vi "Command.vi"(8 "error in (no error)":errorcluster, 9 "command data":u8[](array[numeric]), 10 "node address":u8, 11 "ProPar in":refnum<class "PL Bronkhorst ProPar.lvclass">) -> (0 "error out":errorcluster, 2 "response data":u8[](array[numeric]), 3 "ProPar out":refnum<class "PL Bronkhorst ProPar.lvclass">)   [LabVIEW 2015, in "PL Bronkhorst ProPar.lvclass"]
doc: "Sends specified <b>command data</b> to specified <b>node</b> and returns <b>response data</b>."
uses:
  PL Bronkhorst ProPar.lvclass
  PL Bronkhorst ProPar.lvclass/PL Bronkhorst ProPar.ctl
panel:
  out "response":u8[](array[numeric])
  out "header":u8[](array[numeric])
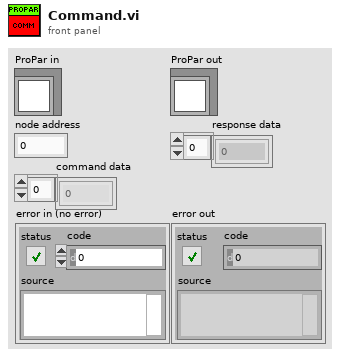
[diagram p1: front panel]
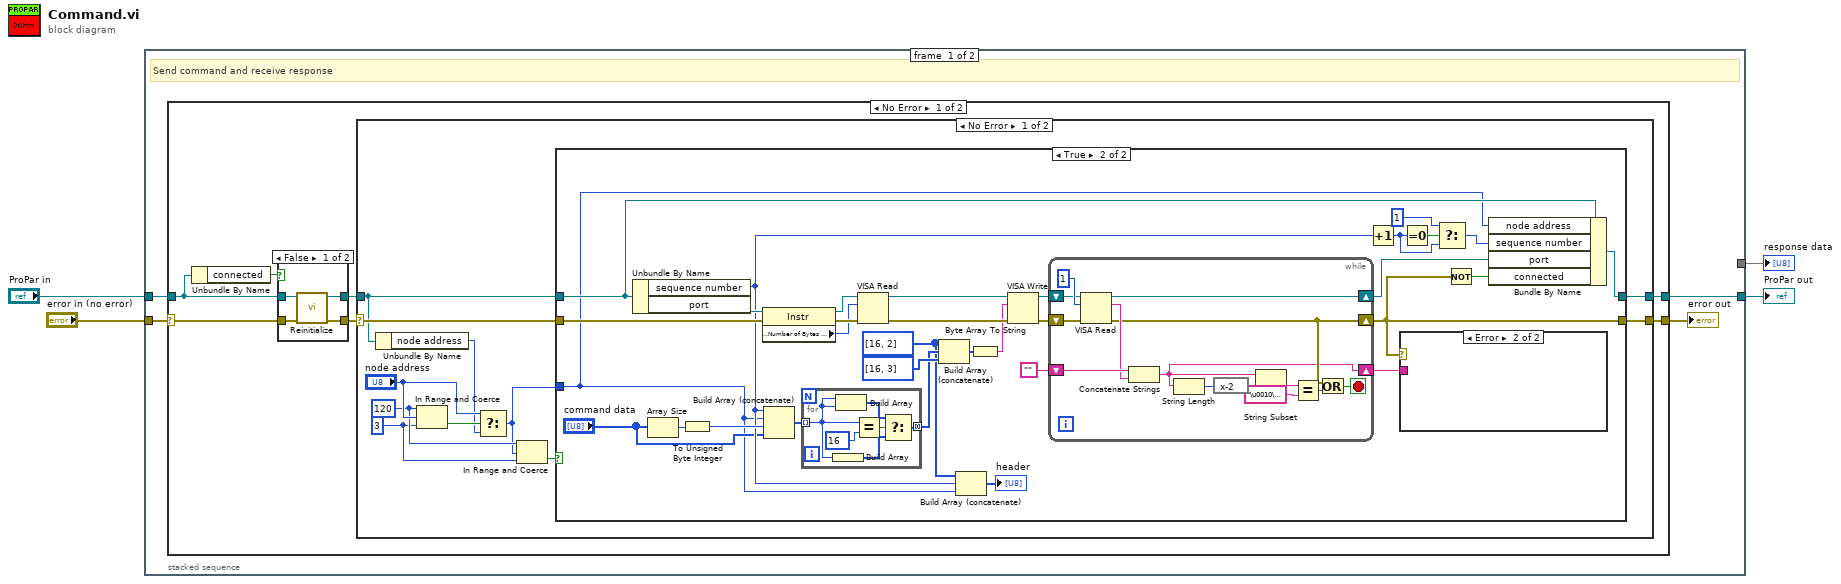
[diagram p0: block diagram]
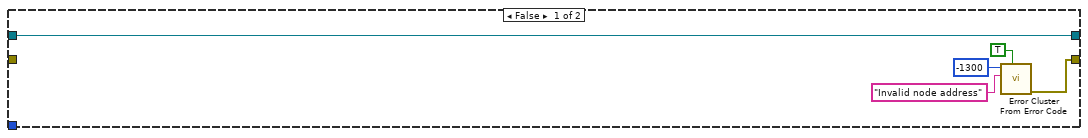
[diagram p2: hidden frame]
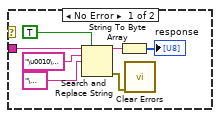
[diagram p3: hidden frame]
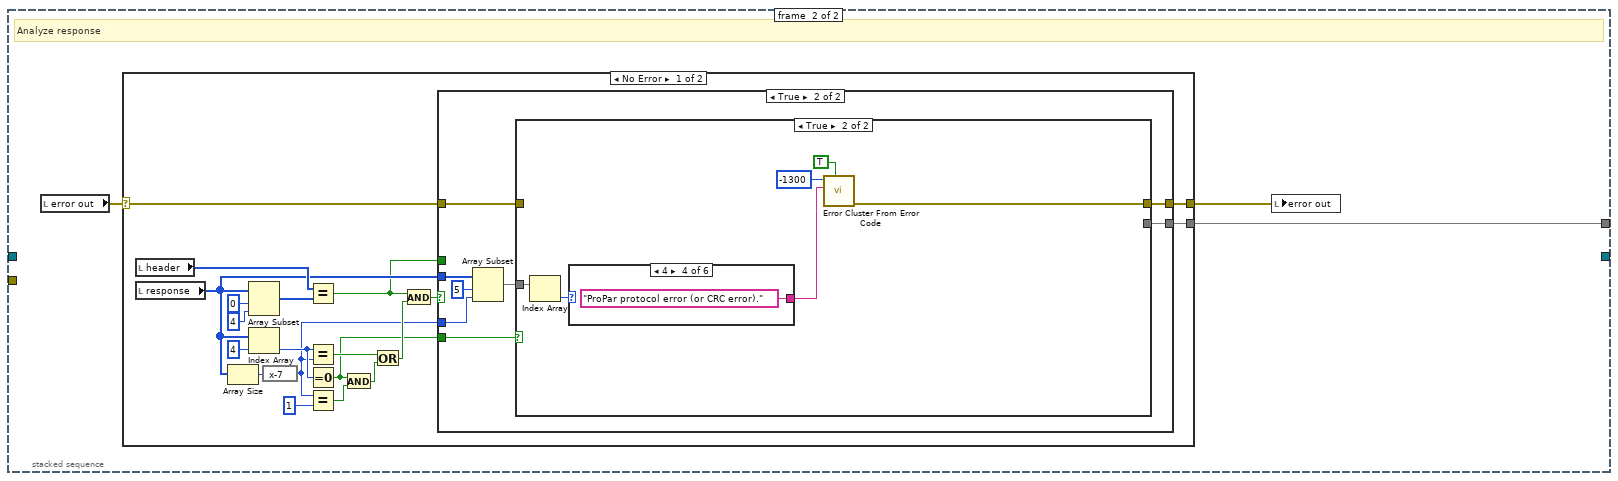
[diagram p7: hidden frame]
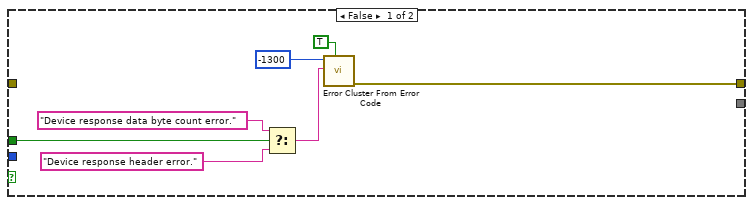
[diagram p8: hidden frame]
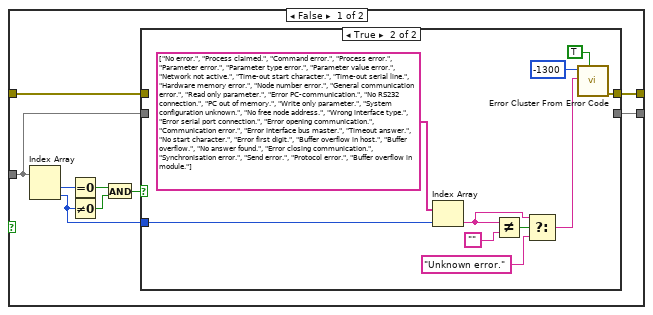
[diagram p9: hidden frame]
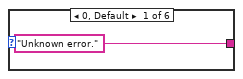
[diagram p11: hidden frame]
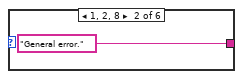
[diagram p12: hidden frame]
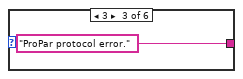
[diagram p13: hidden frame]
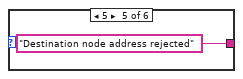
[diagram p14: hidden frame]
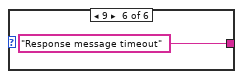
[diagram p15: hidden frame]
diagram:
  n1 = stacked-sequence {
    tunnel: "ProPar in" -> [w8 _]
    tunnel: "error in (no error)" -> [w7 _]
    tunnel: [w6 _] -> w2
    tunnel: [_ w101] -> w1
    frame #0 {
      # "Send command and receive response"
      n2 = case shown="No Error" w7 {
        selector: w7 -> [w13 w100]
        tunnel: w8 -> [w14 w99]
        tunnel: [w10 w100] -> w5
        tunnel: [w9 w99] -> w6
        frame No Error {
          n3 = Unbundle By Name(w14) -> ("connected"=w15:bool)
          n4 = case shown="False" w15 {
            tunnel: w14 -> [w96 w98]
            tunnel: w13 -> [w95 w97]
            tunnel: [w94 w98] -> w11
            tunnel: [w93 w97] -> w12
            frame False {
              n5 = call "Reinitialize.vi"("error in (no error)"=w95, "ProPar in"=w96) -> ("error out"=w93:errorcluster, "ProPar out"=w94:refnum<class "PL Bronkhorst ProPar.lvclass">)  [unwired: 8 in]
            }
            frame True {
            }
          }
          n6 = case shown="No Error" w12 {
            selector: w12 -> [w25 w92]
            tunnel: w11 -> [w21 w91]
            tunnel: [w24 w92] -> w10
            tunnel: [w26 w91] -> w9
            frame No Error {
              w18 = u8 3 ("lower limit")
              w19 = u8 120 ("upper limit")
              n7 = Unbundle By Name(w21) -> ("node address"=w20:u8)
              n8 = In Range and Coerce(upper limit=w19, x="node address", lower limit=w18) -> (In Range?=w23:bool)  [unwired: 1 out]
              n9 = Select(t="node address", s=w23, f=w20) -> (s? t:f=w16:u8)
              n10 = In Range and Coerce(upper limit=w19, x=w16, lower limit=w18) -> (In Range?=w17:bool)  [unwired: 1 out]
              n11 = case shown="True" w17 {
                tunnel: [w31 w63] -> w26
                tunnel: w25 -> [_ w56]
                tunnel: [w27 w36] -> w24
                tunnel: w21 -> [w31 w34]
                tunnel: w16 -> [_ w32]
                frame False {
                  n12 = call <vilib>:"Error Cluster From Error Code.vi"("show call chain? (False)"=TRUE, "error message (\"\")"="Invalid node address" ("format string"), "error code (0)"=-1300) -> ("error out"=w27:errorcluster)  [unwired: 6 in]
                }
                frame True {
                  w39 = u8[] [16, 2]
                  n13 = Unbundle By Name(w34) -> ("sequence number"=w35:u8, "port"=w57:refnum<visa-resource-name>)
                  n14 = Array Size(array="command data") -> (size(s)=w62:i32)
                  n15 = To Unsigned Byte Integer(number=w62) -> (unsigned 8bit integer=w40:u8)
                  n16 = property class="Instr"(reference=w57, error in=w56) -> (reference out=w55:refnum<visa-resource-name>, error out=w54:errorcluster, "Serial Settings:Number of Bytes at Serial Port"=w53:u32)
                  n17 = Build Array (concatenate)(w35, w32, w40, "command data") -> (w41:u8[])
                  n18 = for {
                    tunnel: w41 -> [w87] mode=indexing
                    tunnel: [w85] -> w42 mode=concatenating
                    n19 = Build Array(w87) -> (w88:u8[])
                    n20 = Build Array(w87, w87) -> (w86:u8[])
                    n21 = Equal?(x=w87, y=u8 16) -> (x = y?=w89:bool)
                    n22 = Select(t=w86, s=w89, f=w88) -> (s? t:f=w85:u8[])
                  }
                  n23 = VISA Read(VISA resource name=w55, byte count=w53, error in (no error)=w54) -> (VISA resource name out=w52:refnum<visa-resource-name>, error out=w51:errorcluster)  [unwired: 2 out]
                  n24 = Build Array (concatenate)(w39, w42, u8[] [16, 3]) -> (w50:u8[])
                  n25 = Build Array (concatenate)(w39, w35, w32) -> (→"header":u8[])
                  n26 = Byte Array To String(unsigned byte array=w50) -> (string=w49:string)
                  n27 = VISA Write(VISA resource name=w52, write buffer=w49, error in (no error)=w51) -> (VISA resource name out=w48:refnum<visa-resource-name>, error out=w47:errorcluster)  [unwired: 1 out]
                  n28 = while {
                    shift-right: [w72] -> w36
                    shift-left: w47 -> [w84]
                    shift-right: [w83] -> w46
                    shift-left: w48 -> [w80]
                    shift-right: [w71] -> w37
                    shift-left: "" -> [w79]
                    stop <- w81 stop-if-true
                    n29 = VISA Read(VISA resource name=w80, byte count=u32 1, error in (no error)=w84) -> (VISA resource name out=w83:refnum<visa-resource-name>, read buffer=w78:string, error out=w72:errorcluster)  [unwired: 1 out]
                    n30 = Concatenate Strings(w79, w78) -> (w71:string)
                    n31 = String Length(string=w71) -> (length=w77:i32)
                    n32 = expression code="x-2"(w77) -> (w76:i32)
                    n33 = String Subset(string=w71, offset (0)=w76) -> (substring=w75:string)  [unwired: 1 in]
                    n34 = Equal?(x=w75, y="\u0010\u0003" ("string")) -> (x = y?=w73:bool)
                    n35 = Or(x=w72, y=w73) -> (x .or. y?=w81:bool)
                  }
                  n36 = Increment(x=w35) -> (x+1=w60:u8)
                  n37 = case shown="Error" w36 {
                    tunnel: w37 -> [w65 _]
                    frame No Error {
                      n38 = Search and Replace String(replace all?=TRUE ("replace all? (F)"), input string=w65, search string="\u0010\u0010" ("string"), replace string="\u0010" ("string")) -> (result string=w67:string, error out=w64:errorcluster)  [unwired: 4 in, 2 out]
                      n39 = String To Byte Array(string=w67) -> (unsigned byte array=→"response":u8[])
                      n40 = call <vilib>:"Clear Errors.vi"("error in (no error)"=w64) -> ()  [unwired: 5 in, 2 out]
                    }
                    frame Error {
                    }
                  }
                  n41 = Equal To 0?(x=w60) -> (x = 0?=w61:bool)
                  n42 = Select(t=u8 1, s=w61, f=w60) -> (s? t:f=w58:u8)
                  n43 = Not(x=w36) -> (.not. x?=w45:bool)
                  n44 = Bundle By Name(cluster=w34, "node address"=w32, "sequence number"=w58, "port"=w46, "connected"=w45) -> (w63:refnum<class "PL Bronkhorst ProPar.lvclass">)
                }
              }
            }
            frame Error {
            }
          }
        }
        frame Error {
        }
      }
      "error out" <- w5
    }
    frame #1 {
      # "Analyze response"
      n45 = local read "error out"() -> (w103:errorcluster)
      n46 = case shown="No Error" w103 {
        selector: w103 -> [w108 w172]
        tunnel: [w112 w172] -> w102
        tunnel: [w105 _] -> w101
        frame No Error {
          n47 = local read "header"() -> (w114:u8[])
          n48 = local read "response"() -> (w107:u8[])
          n49 = Array Size(array=w107) -> (size(s)=w118:i32)
          n50 = Array Subset(array=w107, index=0, length=4) -> (w111:u8[])
          n51 = Index Array(array=w107, index=4) -> (element=w109:u8)
          n52 = expression code="x-7"(w118) -> (w106:i32)
          n53 = Equal?(x=w114, y=w111) -> (x = y?=w104:bool)
          n54 = Equal?(x=w109, y=w106) -> (x = y?=w120:bool)
          n55 = Equal To 0?(x=w109) -> (x = 0?=w110:bool)
          n56 = Equal?(x=w106, y=1) -> (x = y?=w122:bool)
          n57 = And(x=w110, y=w122) -> (x .and. y?=w123:bool)
          n58 = Or(x=w120, y=w123) -> (x .or. y?=w119:bool)
          n59 = And(x=w104, y=w119) -> (x .and. y?=w113:bool)
          n60 = case shown="True" w113 {
            tunnel: [w128 w137] -> w112
            tunnel: w107 -> [_ w136]
            tunnel: w110 -> [_ w138]
            tunnel: w106 -> [_ w134]
            tunnel: w108 -> [_ w132]
            tunnel: [_ w131] -> w105
            tunnel: w104 -> [w126 _]
            frame False {
              n61 = Select(t="Device response data byte count error." ("format string"), s=w126, f="Device response header error." ("format string")) -> (s? t:f=w124:string)
              n62 = call <vilib>:"Error Cluster From Error Code.vi"("show call chain? (False)"=TRUE, "error message (\"\")"=w124, "error code (0)"=-1300) -> ("error out"=w128:errorcluster)  [unwired: 6 in]
            }
            frame True {
              n63 = Array Subset(array=w136, index=5, length=w134) -> (w133:u8[])
              n64 = case shown="True" w138 {
                tunnel: [w142 w162] -> w137
                tunnel: w133 -> [w140 w161]
                tunnel: w132 -> [w141 _]
                tunnel: [w139 _] -> w131
                frame False {
                  n65 = Index Array(array=w140) -> (element #1=w147:u8, element #2=w143:u8)  [unwired: 2 in]
                  n66 = Equal To 0?(x=w147) -> (x = 0?=w146:bool)
                  n67 = Not Equal To 0?(x=w143) -> (x != 0?=w145:bool)
                  n68 = And(x=w146, y=w145) -> (x .and. y?=w144:bool)
                  n69 = case shown="True" w144 {
                    tunnel: w143 -> [_ w155]
                    tunnel: [w149 w157] -> w142
                    tunnel: w141 -> [w149 _]
                    tunnel: w140 -> [w148 _]
                    tunnel: [w148 _] -> w139
                    frame False {
                    }
                    frame True {
                      n70 = Index Array(array=string[] ["No error.", "Process claimed.", "Command error.", "Process error.", "Parameter error.", "Parameter type error.", "Parameter value error.", "Network not active.", "Time-out start character.", "Time-out serial line.", "Hardware memory error.", "Node number error.", "General communication error.", "Read only parameter.", "Error PC-communication.", "No RS232 connection.", "PC out of memory.", "Write only parameter.", "System configuration unknown.", "No free node address.", "Wrong interface type.", "Error serial port connection.", "Error opening communication.", "Communication error.", "Error interface bus master.", "Timeout answer.", "No start character.", "Error first digit.", "Buffer overflow in host.", "Buffer overflow.", "No answer found.", "Error closing communication.", "Synchronisation error.", "Send error.", "Protocol error.", "Buffer overflow in module."], index=w155) -> (element=w152:string)
                      n71 = Not Equal?(x=w152, y="") -> (x != y?=w153:bool)
                      n72 = Select(t=w152, s=w153, f="Unknown error.") -> (s? t:f=w150:string)
                      n73 = call <vilib>:"Error Cluster From Error Code.vi"("show call chain? (False)"=TRUE, "error message (\"\")"=w150, "error code (0)"=-1300) -> ("error out"=w157:errorcluster)  [unwired: 6 in]
                    }
                  }
                }
                frame True {
                  n74 = Index Array(array=w161) -> (element=w160:u8)  [unwired: 1 in]
                  n75 = case shown="4" w160 {
                    tunnel: ["Unknown error." ("format string") "General error." ("format string") "ProPar protocol error." ("format string") "ProPar protocol error (or CRC error)." ("format string") "Destination node address rejected" ("format string") "Response message timeout" ("format string")] -> w163
                    frame 0, Default {
                    }
                    frame 1, 2, 8 {
                    }
                    frame 3 {
                    }
                    frame 4 {
                    }
                    frame 5 {
                    }
                    frame 9 {
                    }
                  }
                  n76 = call <vilib>:"Error Cluster From Error Code.vi"("show call chain? (False)"=TRUE, "error message (\"\")"=w163, "error code (0)"=-1300) -> ("error out"=w162:errorcluster)  [unwired: 6 in]
                }
              }
            }
          }
        }
        frame Error {
        }
      }
      n77 = local write "error out"(w102) -> ()
    }
  }
  "ProPar out" <- w2
  "response data" <- w1
